vi "Read Test Info.vi"(8 "error in (no error)":errorcluster, 11 "CSL configuration":refnum<class "CSL configuration.lvclass">) -> (0 "error out":errorcluster, 2 "Test Info":T1={"General"={"Operator"="JLee"}}, 3 "CSL configuration out":refnum<class "CSL configuration.lvclass">)   [LabVIEW 2025, in "CSL.lvlib" / "CSL configuration.lvclass"]
uses:
  CSL configuration.lvclass
  Test Info.ctl
  CSL configuration.lvclass/CSL configuration.ctl
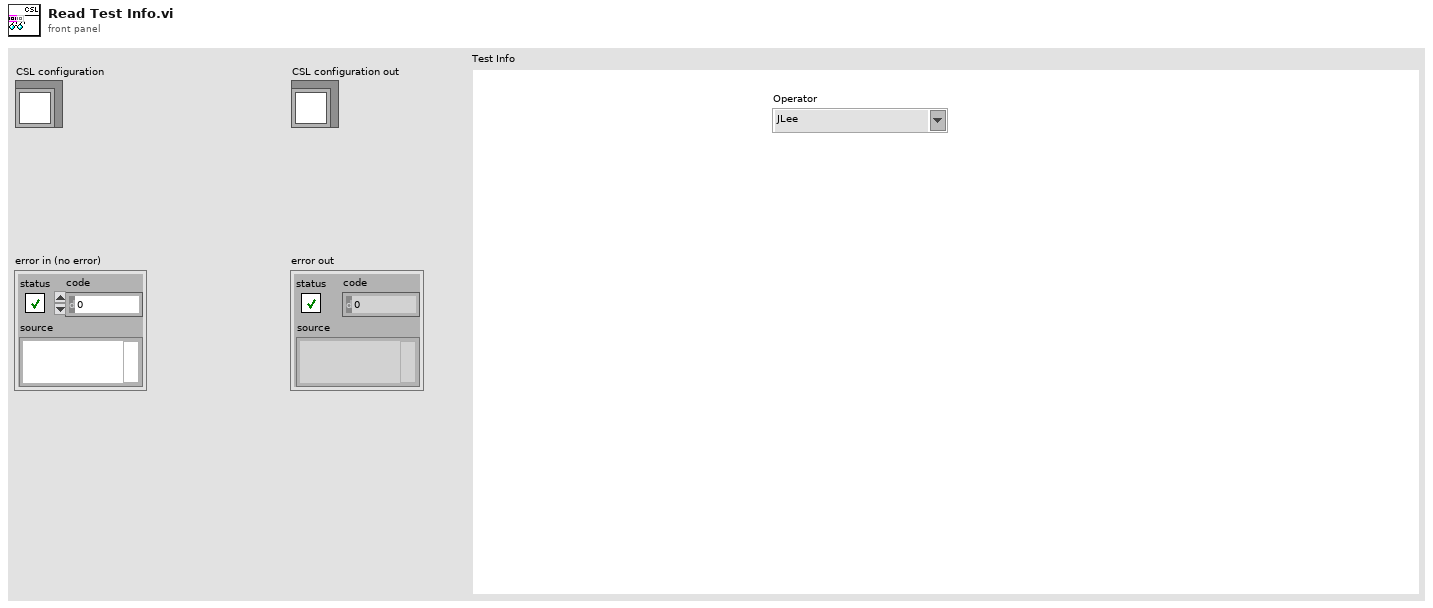
[diagram p1: front panel]
types:
  T1 = typedef "CSL.lvlib/CSL configuration.lvclass/Test Info.ctl" = cluster{"General":cluster{"Operator":string}}
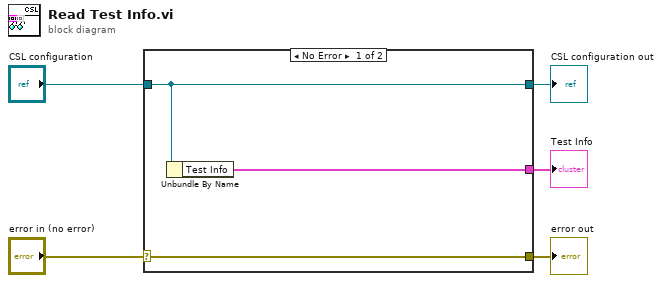
[diagram p0: block diagram]
diagram:
  n1 = case shown="No Error" "error in (no error)" {
    selector: "error in (no error)" -> [w8 w9]
    tunnel: [w8 w9] -> w4
    tunnel: [w7 w10] -> w1
    tunnel: "CSL configuration" -> [w7 w10]
    tunnel: [w6 _] -> w3
    frame No Error {
      n2 = Unbundle By Name(w7) -> ("Test Info"=w6:T1)
    }
    frame Error {
    }
  }
  "error out" <- w4
  "Test Info" <- w3
  "CSL configuration out" <- w1
